vi "AlliGator Panel VI Name.vi"(11 "Panel VI Name":string) -> (3 "Panel Name":string)   [LabVIEW 2021, in "AlliGator GUI.lvlib"]
uses:
  AlliGator GUI.lvlib
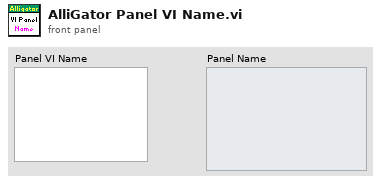
[diagram p1: front panel]
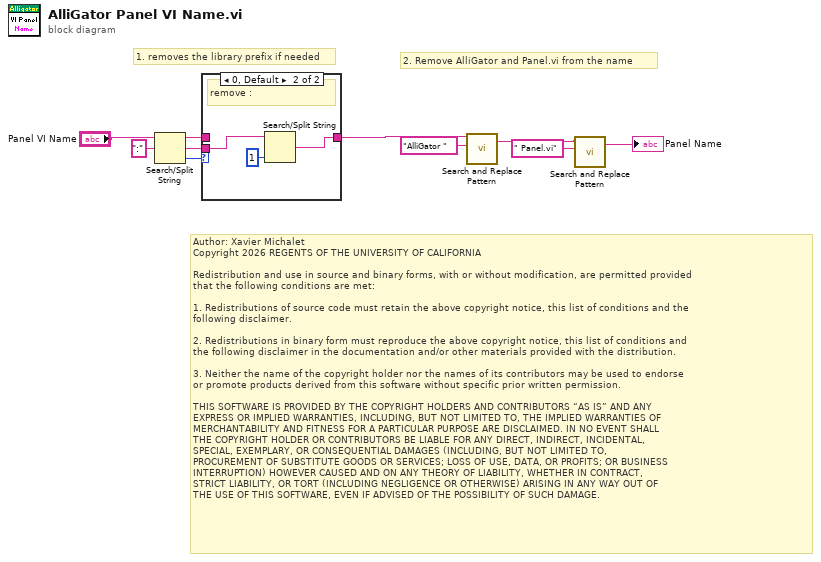
[diagram p0: block diagram]
diagram:
  # "2. Remove AlliGator and Panel.vi from the name"
  # "1. removes the library prefix if needed"
  # "Author: Xavier Michalet\nCopyright 2026 REGENTS OF THE UNIVERSITY OF CALIFORNIA\n\nRedistribution and use in source and binary forms, with or without modification, are permitted provided\nthat the following conditions are met:\n\n1. Redistributions of source code must retain the above copyright notice, this list of conditions and the\nfollowing disclaimer.\n\n2. Redistributions in binary form must reproduce the above copyright notice, this list of conditions and\nthe following disclaimer in the documentation and/or other materials provided with the distribution.\n\n3. Neither the name of the copyright holder nor the names of its contributors may be used to endorse \nor promote products derived from this software without specific prior written permission.\n\nTHIS SOFTWARE IS PROVIDED BY THE COPYRIGHT HOLDERS AND CONTRIBUTORS “AS IS” AND ANY \nEXPRESS OR IMPLIED WARRANTIES, INCLUDING, BUT NOT LIMITED TO, THE IMPLIED WARRANTIES OF\nMERCHANTABILITY AND FITNESS FOR A PARTICULAR PURPOSE ARE DISCLAIMED. IN NO EVENT SHALL\nTHE COPYRIGHT HOLDER OR CONTRIBUTORS BE LIABLE FOR ANY DIRECT, INDIRECT, INCIDENTAL, \nSPECIAL, EXEMPLARY, OR CONSEQUENTIAL DAMAGES (INCLUDING, BUT NOT LIMITED TO, \nPROCUREMENT OF SUBSTITUTE GOODS OR SERVICES; LOSS OF USE, DATA, OR PROFITS; OR BUSINESS\nINTERRUPTION) HOWEVER CAUSED AND ON ANY THEORY OF LIABILITY, WHETHER IN CONTRACT, \nSTRICT LIABILITY, OR TORT (INCLUDING NEGLIGENCE OR OTHERWISE) ARISING IN ANY WAY OUT OF\nTHE USE OF THIS SOFTWARE, EVEN IF ADVISED OF THE POSSIBILITY OF SUCH DAMAGE."
  n1 = Search/Split String(string="Panel VI Name", search string/char (-)=":") -> (substring before match=w1:string, match + rest of string=w5:string, offset of match=w2:i32)  [unwired: 1 in]
  n2 = case shown="0, Default" w2 {
    tunnel: w5 -> [_ w14]
    tunnel: [w11 w12] -> w3
    tunnel: w1 -> [w11 _]
    frame -1 {
    }
    frame 0, Default {
      # "remove :"
      n3 = Search/Split String(string=w14, offset (0)=1) -> (match + rest of string=w12:string)  [unwired: 1 in, 2 out]
    }
  }
  n4 = call <vilib>:"Search and Replace Pattern.vi"("string"=w3, "regular expression (\"\")"="AlliGator " ("regular expression (\"\")")) -> ("result string"=w8:string)  [unwired: 3 in, 1 out]
  n5 = call <vilib>:"Search and Replace Pattern.vi"("string"=w8, "regular expression (\"\")"=" Panel.vi" ("regular expression (\"\")")) -> ("result string"=→"Panel Name":string)  [unwired: 3 in, 1 out]
